vi "Deserialize Data in Wrapper.vi"(0 "VI in":refnum<vi>, 5 "Terms[]":refnum<vi>[](array[refnum]), 7 "Control Names":string[](array[string]), 11 "error in (no error)":errorcluster) -> (15 "error out":errorcluster)   [LabVIEW 2021, in "Migrator.lvlib"]
uses:
  Migrator.lvlib
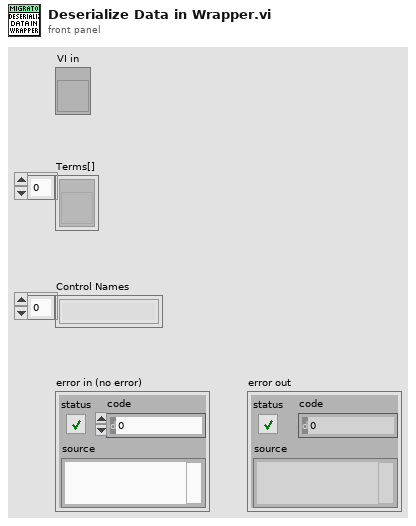
[diagram p1: front panel]
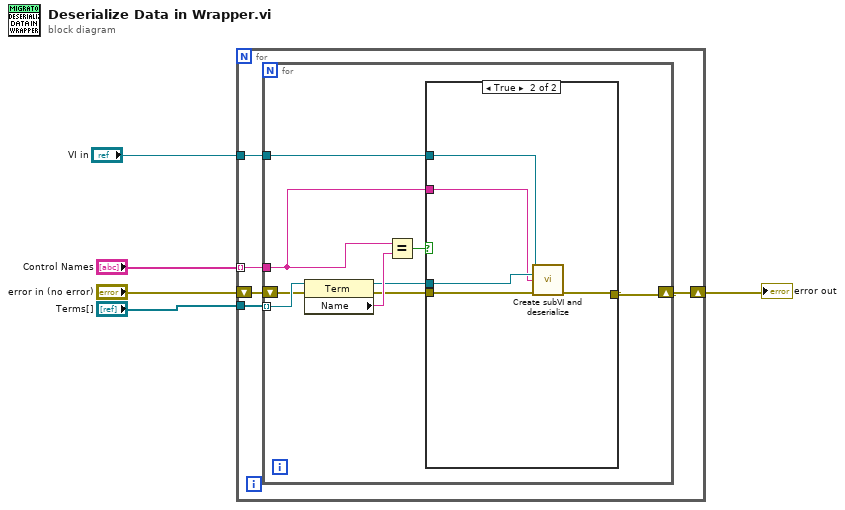
[diagram p0: block diagram]
diagram:
  n1 = for {
    tunnel: "Terms[]" -> [w10]
    tunnel: "Control Names" -> [w8] mode=indexing
    shift-right: [w6] -> w4
    shift-left: "error in (no error)" -> [w9]
    tunnel: "VI in" -> [w7]
    n2 = for {
      tunnel: w10 -> [w19] mode=indexing
      shift-right: [w12] -> w6
      shift-left: w9 -> [w17]
      tunnel: w8 -> [w11]
      tunnel: w7 -> [w13]
      n3 = property class="Term"(reference=w19, error in=w17) -> (reference out=w14:refnum<vi>, error out=w15:errorcluster, "Name"=w18:string)
      n4 = Equal?(x=w11, y=w18) -> (x = y?=w16:bool)
      n5 = case shown="True" w16 {
        tunnel: w15 -> [w20 w24]
        tunnel: w14 -> [_ w25]
        tunnel: w13 -> [_ w23]
        tunnel: [w20 w21] -> w12
        tunnel: w11 -> [_ w22]
        frame False {
        }
        frame True {
          n6 = call "Create subVI and deserialize.vi"("VI in"=w23, "Term Refnum"=w25, "Name Out"=w22, "error in (no error)"=w24) -> ("error out"=w21:errorcluster)  [unwired: 11 in]
        }
      }
    }
  }
  "error out" <- w4
